vi "PSGetPngChunks.vi"(11 "data":string) -> (0 "CRC":string[](array[string]), 1 "Data":string[](array[string]), 2 "Name":string[](array[string]), 3 "Length":u32[](array[numeric]), 4 "Chunks":string[](array[string]), 5 "Header":string)   [LabVIEW 2013, in "VIVendor.lvlib" / "VVPngSnippet.lvlib"]
doc: "Retrieves all chunks from a PNG file.\nCreated by Darin\n\nOrigin:\n* PNG Snippet VIs from Code Complete Tool\n* http://sourceforge.net/projects/lv-cct-tool/\n* Commit: 9d97aea5cbd2fc456c5914801e927df6a901d523\n* License: BSD -- see NOTICE.txt"
uses:
  VVPngSnippet.lvlib
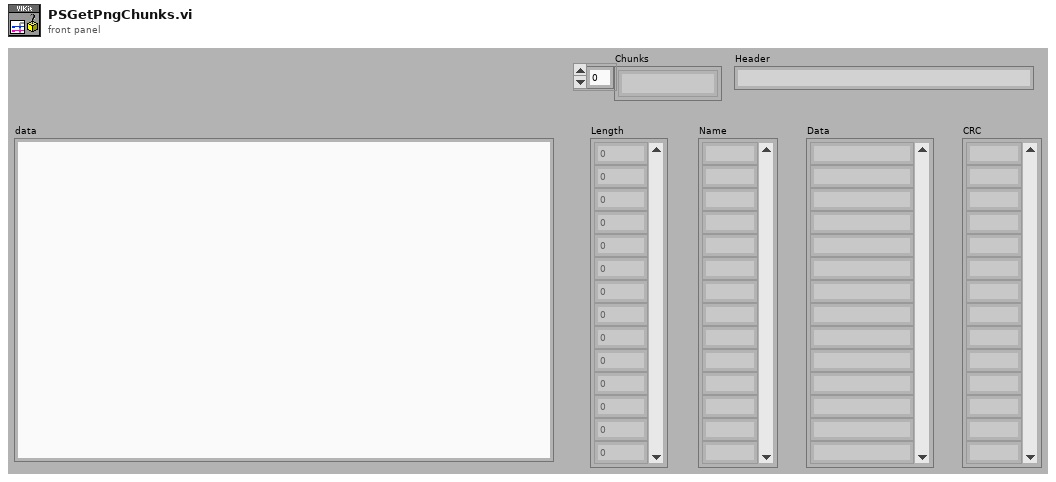
[diagram p1: front panel]
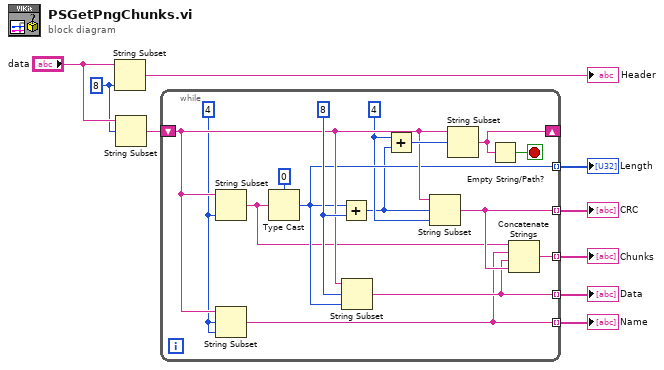
[diagram p0: block diagram]
diagram:
  w1 = 8 ("length (rest)")
  n1 = String Subset(string="data", length (rest)=w1) -> (substring=→"Header":string)  [unwired: 1 in]
  n2 = String Subset(string="data", offset (0)=w1) -> (substring=w2:string)  [unwired: 1 in]
  n3 = while {
    shift-right: [w18] -> _
    shift-left: w2 -> [w21]
    tunnel: [w19] -> w9 mode=indexing
    tunnel: [w16] -> w7 mode=indexing
    tunnel: [w17] -> w6 mode=indexing
    tunnel: [w15] -> w8 mode=indexing
    tunnel: [w13] -> w5 mode=indexing
    stop <- w20 stop-if-true
    w11 = 4 ("length (rest)")
    w23 = 8 ("offset (0)")
    w12 = 4 ("length (rest)")
    n4 = String Subset(string=w21, length (rest)=w12) -> (substring=w14:string)  [unwired: 1 in]
    n5 = String Subset(string=w21, offset (0)=w12, length (rest)=w12) -> (substring=w15:string)
    n6 = Type Cast(type=u32 0, x=w14) -> (*(type *) &x=w19:u32)
    n7 = Add(x=w19, y=w23) -> (x+y=w10:u32)
    n8 = String Subset(string=w21, offset (0)=w23, length (rest)=w19) -> (substring=w16:string)
    n9 = Add(x=w11, y=w10) -> (x+y=w22:u32)
    n10 = String Subset(string=w21, offset (0)=w10, length (rest)=w11) -> (substring=w17:string)
    n11 = String Subset(string=w21, offset (0)=w22) -> (substring=w18:string)  [unwired: 1 in]
    n12 = Empty String/Path?(string/path=w18) -> (empty?=w20:bool)
    n13 = Concatenate Strings(w14, w15, w16, w17) -> (w13:string)
  }
  "Length" <- w9
  "Name" <- w8
  "Data" <- w7
  "CRC" <- w6
  "Chunks" <- w5
